vi "Create Message Setter (from Accessor).vi"(8 "error in (no error)":errorcluster, 10 "RPC Message Name":string, 11 "RPC Messages Folder (ProjectItem) in":refnum<vi>) -> (0 "error out":errorcluster, 1 "Created ?":bool, 2 "Setter VI out":refnum<vi>, 3 "RPC Messages Folder (ProjectItem) out":refnum<vi>)   [LabVIEW 2019, in "gRPC Template Creation Utility.lvlib"]
uses:
  gRPC Template Creation Utility.lvlib
  TypeDefs/Method Accessor Type.ctl
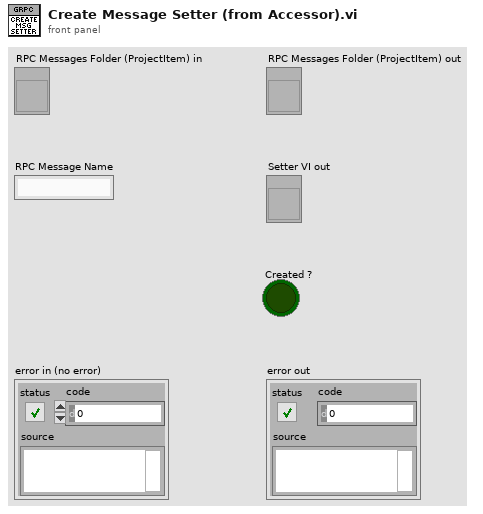
[diagram p1: front panel]
types:
  T1 = typedef "gRPC Template Creation Utility.lvlib/Method Accessor Type.ctl" = string
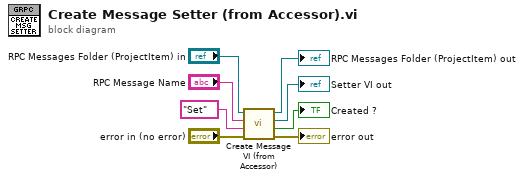
[diagram p0: block diagram]
diagram:
  n1 = call "Create Message VI (from Accessor).vi"("error in (no error)"="error in (no error)", "accessor type"=T1 "Set", "rpc message name"="RPC Message Name", "rpc messages folder in"="RPC Messages Folder (ProjectItem) in") -> ("error out"=→"error out":errorcluster, "created?"=→"Created ?":bool, "accessor vi"=→"Setter VI out":refnum<vi>, "rpc messages folder out"=→"RPC Messages Folder (ProjectItem) out":refnum<vi>)  [unwired: 4 in]
